vi "test tools list array items.vi"(8 "error in (no error)":errorcluster) -> (0 "error out":errorcluster, 3 "body":string)   [LabVIEW 2020, in "MCP Server tests.lvlib"]
doc: "tools/list must describe an array input with items and the type of its elements."
uses:
  MCP Server tests.lvlib
  <vilib>/JDP Science/JSONtext/Next JSON Value.vi
  <vilib>/JDP Science/JSONtext/String Subset.vi
  <vilib>/JDP Science/JSONtext/Parsing/Advance past next JSON Value (inlined COPY).vi
  <vilib>/JDP Science/JSONtext/Parsing/Advance past whitespace.vi
  <vilib>/JDP Science/JSONtext/Parsing/Advance past String.vi
  <vilib>/JDP Science/JSONtext/Parsing/Advance past Number.vi
  <vilib>/JDP Science/JSONtext/Parsing/Advance past Line Ending.vi
  <vilib>/JDP Science/JSONtext/Parsing/Parse Full Path or Item Name.vi
  <vilib>/JDP Science/JSONtext/Parsing/Advance past Array.vi
  <vilib>/JDP Science/JSONtext/Parsing/Advance past Object.vi
  <vilib>/JDP Science/JSONtext/support/Error Cluster From Code.vi
  <vilib>/JDP Science/JSONtext/Offset/Find Item Locations by Path.vi
  <vilib>/addons/_JKI Toolkits/Caraya/classes/Test/Test.lvclass
  <vilib>/JDP Science/JSONtext/JSONtext.lvlib
  <vilib>/addons/_JKI Toolkits/Caraya/classes/Assert/Assert.lvclass
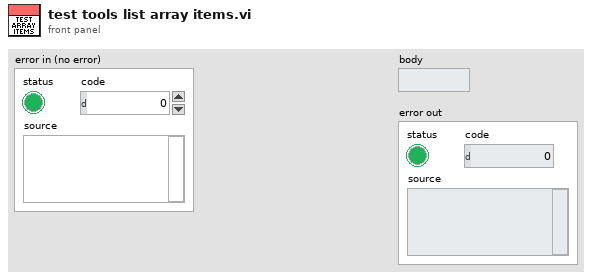
[diagram p1: front panel]
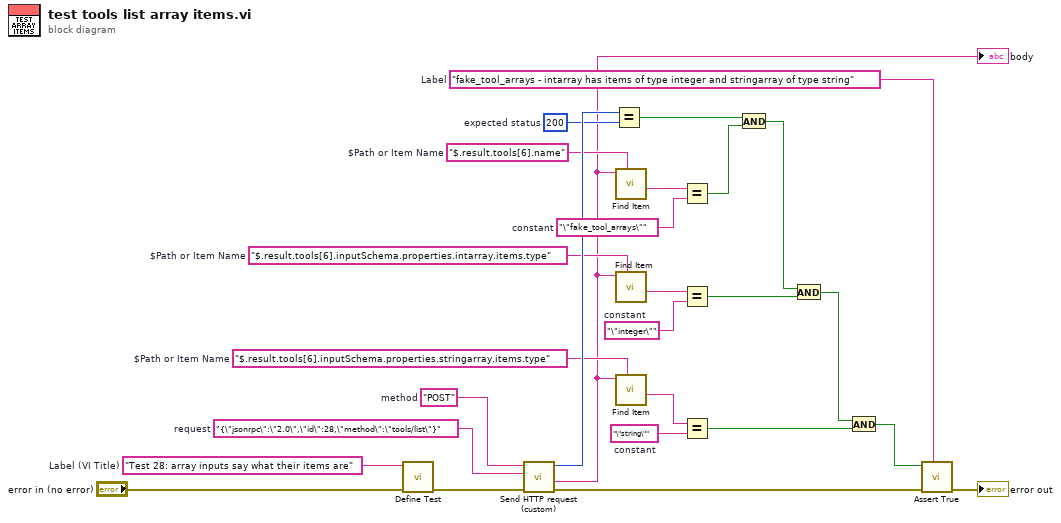
[diagram p0: block diagram]
diagram:
  w3 = "fake_tool_arrays - intarray has items of type integer and stringarray of type string"  # Label
  w12 = "\"string\""  # constant
  w14 = "\"integer\""  # constant
  w16 = "\"fake_tool_arrays\""  # constant
  w18 = "$.result.tools[6].inputSchema.properties.stringarray.items.type"  # $Path or Item Name
  w19 = "$.result.tools[6].inputSchema.properties.intarray.items.type"  # $Path or Item Name
  w20 = "$.result.tools[6].name"  # $Path or Item Name
  w21 = 200  # expected status
  w24 = "{\"jsonrpc\":\"2.0\",\"id\":28,\"method\":\"tools/list\"}"  # request
  w25 = "POST"  # method
  w27 = "Test 28: array inputs say what their items are"  # Label (VI Title)
  n1 = call <vilib>:"Define Test.vi"("error in (no error)"="error in (no error)", "Label (VI Title)"=w27) -> ("error out"=w23:errorcluster)  [unwired: 8 in, 1 out]
  n2 = call "Send HTTP request (custom).vi"("error in (no error)"=w23, "request"=w24, "method"=w25) -> ("error out"=w4:errorcluster, "response"=w2:string, "status code"=w22:i32)  [unwired: 5 in, 1 out]
  "body" <- w2
  n3 = Equal?(x=w22, y=w21) -> (x = y?=w11:bool)
  n4 = call <vilib>:"Find Item.vi"("$Path or Item Name"=w20, "JSON"=w2) -> ("<JSON>"=w17:string)  [unwired: 6 in, 3 out]
  n5 = call <vilib>:"Find Item.vi"("$Path or Item Name"=w19, "JSON"=w2) -> ("<JSON>"=w15:string)  [unwired: 6 in, 3 out]
  n6 = call <vilib>:"Find Item.vi"("$Path or Item Name"=w18, "JSON"=w2) -> ("<JSON>"=w13:string)  [unwired: 6 in, 3 out]
  n7 = Equal?(x=w17, y=w16) -> (x = y?=w10:bool)
  n8 = Equal?(x=w15, y=w14) -> (x = y?=w8:bool)
  n9 = Equal?(x=w13, y=w12) -> (x = y?=w6:bool)
  n10 = And(x=w11, y=w10) -> (x .and. y?=w9:bool)
  n11 = And(x=w9, y=w8) -> (x .and. y?=w7:bool)
  n12 = And(x=w7, y=w6) -> (x .and. y?=w5:bool)
  n13 = call <vilib>:"Assert True.vi"("Label"=w3, "error in (no error)"=w4, "True?"=w5) -> ("error out"=→"error out":errorcluster)  [unwired: 7 in, 1 out]
